vi "data_sim.vi"() -> ()   [LabVIEW 2021]
panel:
  in  "Stop 2":bool
  out "길이 2":i32
  out "연결된 문자열 2":string
  out "CRC-CCITT 2":u16 format="%x"
  out "CRC-CCITT":u16 format="%x"
  out "연결된 문자열":string
  out "길이":i32
  in  "Stop":bool
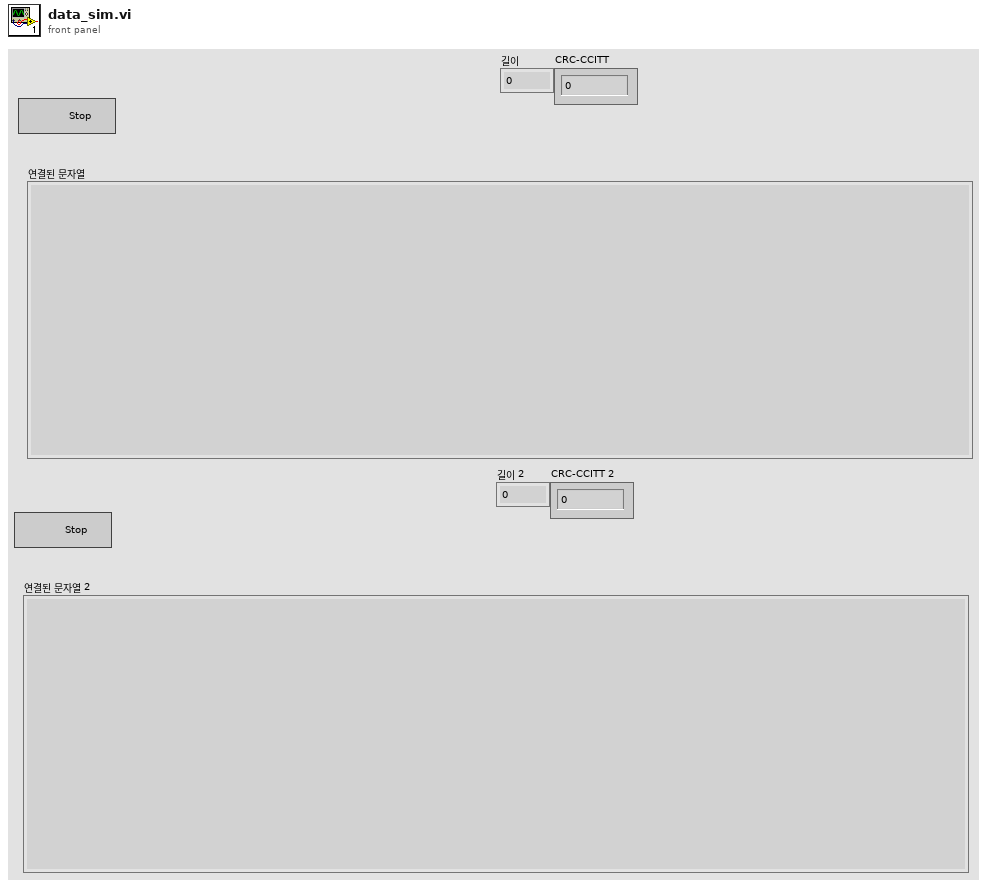
[diagram p1: front panel]
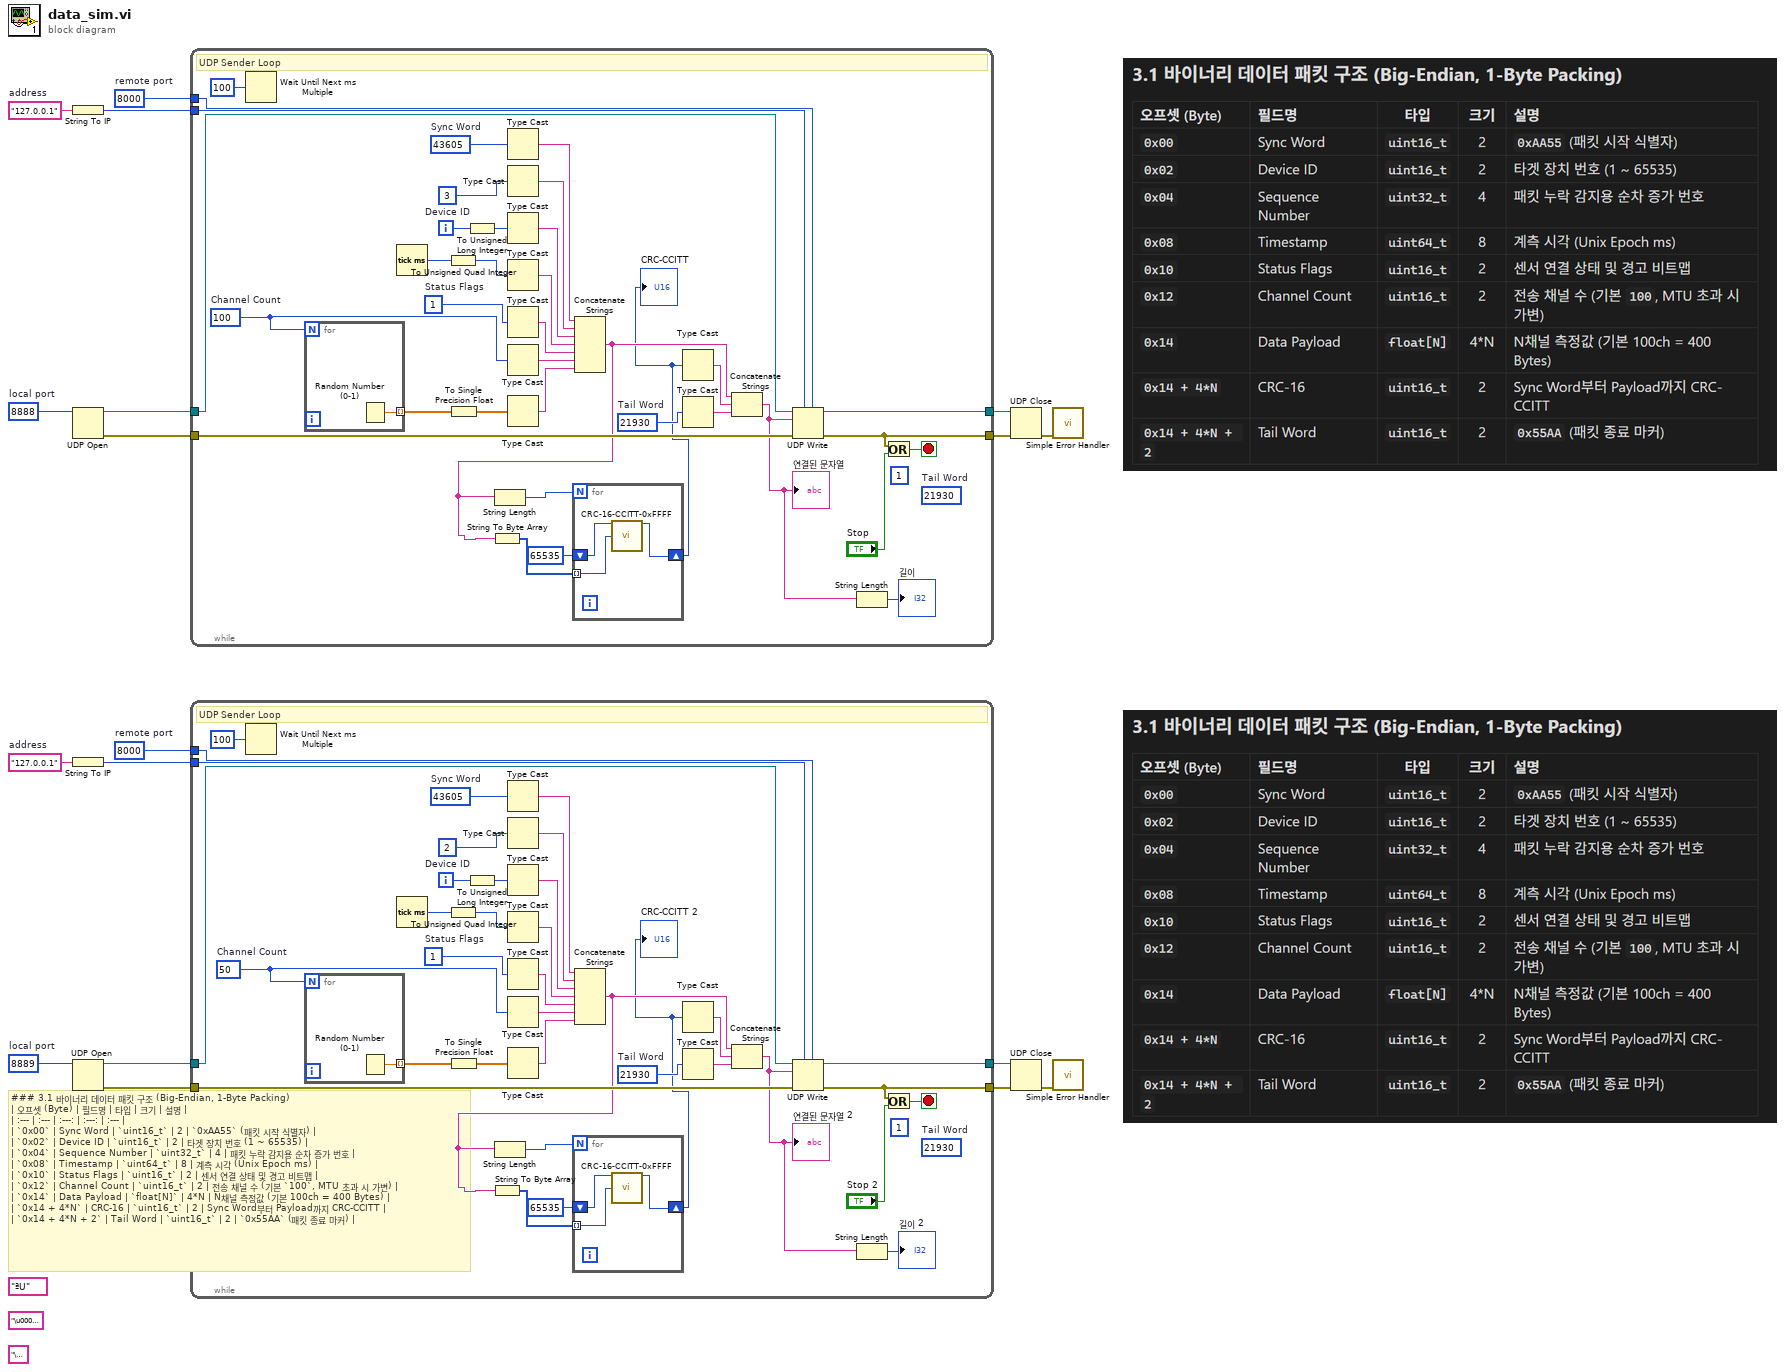
[diagram p0: block diagram]
diagram:
  w9 = u16 8000  # remote port
  w8 = u16 8889  # local port
  w3 = "127.0.0.1"  # address
  (unwired) "\u0001"
  (unwired) "\u0000\u0001"
  (unwired) "ªU"
  w10 = u16 8000  # remote port
  w11 = u16 8888  # local port
  w16 = "127.0.0.1"  # address
  # "### 3.1 바이너리 데이터 패킷 구조 (Big-Endian, 1-Byte Packing)\n| 오프셋 (Byte) | 필드명 | 타입 | 크기 | 설명 |\n| :--- | :--- | :---: | :---: | :--- |\n| `0x00` | Sync Word | `uint16_t` | 2 | `0xAA55` (패킷 시작 식별자) |\n| `0x02` | Device ID | `uint16_t` | 2 | 타겟 장치 번호 (1 ~ 65535) |\n| `0x04` | Sequence Number | `uint32_t` | 4 | 패킷 누락 감지용 순차 증가 번호 |\n| `0x08` | Timestamp | `uint64_t` | 8 | 계측 시각 (Unix Epoch ms) |\n| `0x10` | Status Flags | `uint16_t` | 2 | 센서 연결 상태 및 경고 비트맵 |\n| `0x12` | Channel Count | `uint16_t` | 2 | 전송 채널 수 (기본 `100`, MTU 초과 시 가변) |\n| `0x14` | Data Payload | `float[N]` | 4*N | N채널 측정값 (기본 100ch = 400 Bytes) |\n| `0x14 + 4*N` | CRC-16 | `uint16_t` | 2 | Sync Word부터 Payload까지 CRC-CCITT |\n| `0x14 + 4*N + 2` | Tail Word | `uint16_t` | 2 | `0x55AA` (패킷 종료 마커) |"
  n1 = String To IP(1:w16) -> (0:w14:u32)
  n2 = UDP Open(11:w11) -> (port=w13:refnum<k16>, 0:w12:errorcluster)  [unwired: 4 in, 1 out]
  n3 = String To IP(1:w3) -> (0:w5:u32)
  n4 = UDP Open(11:w8) -> (port=w6:refnum<k16>, 0:w7:errorcluster)  [unwired: 4 in, 1 out]
  n5 = while {
    tunnel: [w49] -> w17
    tunnel: w13 -> [w54]
    tunnel: w12 -> [w53]
    tunnel: [w50] -> w18
    tunnel: w14 -> [w48]
    tunnel: w10 -> [w46]
    i -> [w25]
    stop <- w52 stop-if-true
    w43 = u16 21930  # Tail Word
    (unwired) u16 21930  # Tail Word
    w36 = u16 100  # Channel Count
    w37 = u16 1  # Status Flags
    (unwired) u16 1
    w39 = u16 3  # Device ID
    w40 = u16 43605  # Sync Word
    # "UDP Sender Loop"
    n6 = Wait Until Next ms Multiple(millisecond multiple=u32 100 ("milliseconds to wait")) -> ()  [unwired: 1 out]
    n7 = for {
      N: w36 -> [_]
      tunnel: [w58] -> w44 mode=indexing
      n8 = Random Number (0-1)() -> (number: 0 to 1=w58:dbl)
    }
    n9 = Tick Count (ms)() -> (millisecond timer value=w45:u32)
    n10 = To Unsigned Quad Integer(1:w45) -> (0:w38:u64)
    n11 = To Single Precision Float(number=w44) -> (single precision float=w41:sgl[])
    n12 = To Unsigned Long Integer(number=w25) -> (unsigned 32bit integer=w24:u32)
    n13 = Type Cast(x=w40) -> (*(type *) &x=w30:string)  [unwired: 1 in]
    n14 = Type Cast(x=w39) -> (*(type *) &x=w31:string)  [unwired: 1 in]
    n15 = Type Cast(x=w24) -> (*(type *) &x=w32:string)  [unwired: 1 in]
    n16 = Type Cast(x=w38) -> (*(type *) &x=w33:string)  [unwired: 1 in]
    n17 = Type Cast(x=w37) -> (*(type *) &x=w34:string)  [unwired: 1 in]
    n18 = Type Cast(x=w36) -> (*(type *) &x=w35:string)  [unwired: 1 in]
    n19 = Type Cast(x=w41) -> (*(type *) &x=w27:string)  [unwired: 1 in]
    n20 = Concatenate Strings(w30, w31, w32, w33, w34, w35, w27) -> (w20:string)
    n21 = String To Byte Array(string=w20) -> (unsigned byte array=w23:u8[])
    n22 = String Length(string=w20) -> (length=w22:i32)
    n23 = for {
      N: w22 -> [_]
      tunnel: w23 -> [w56] mode=indexing
      shift-right: [w55] -> w19
      shift-left: u16 65535 ("CRC") -> [w57]
      n24 = call "CRC-16-CCITT-0xFFFF.vi"("CRC In"=w57, "Data"=w56) -> ("CRC"=w55:u16)  [unwired: 12 in, 1 out]
    }
    "CRC-CCITT" <- w19
    n25 = Type Cast(x=w19) -> (*(type *) &x=w29:string)  [unwired: 1 in]
    n26 = Type Cast(x=w43) -> (*(type *) &x=w28:string)  [unwired: 1 in]
    n27 = Concatenate Strings(w20, w29, w28) -> (w26:string)
    "연결된 문자열" <- w26
    n28 = UDP Write(address=w48, port or service name=w46, connection ID=w54, data in=w26, 8:w53) -> (error out=w49:errorcluster, 3:w50:refnum<k16>)  [unwired: 1 in]
    n29 = String Length(string=w26) -> (length=→"길이":i32)
    n30 = Or(x=w49, y="Stop") -> (x .or. y?=w52:bool)
  }
  n31 = while {
    tunnel: [w89] -> w2
    tunnel: w6 -> [w94]
    tunnel: w7 -> [w93]
    tunnel: [w90] -> w1
    tunnel: w5 -> [w88]
    tunnel: w9 -> [w86]
    i -> [w65]
    stop <- w92 stop-if-true
    w83 = u16 21930  # Tail Word
    (unwired) u16 21930  # Tail Word
    w76 = u16 50  # Channel Count
    w77 = u16 1  # Status Flags
    (unwired) u16 1
    w79 = u16 2  # Device ID
    w80 = u16 43605  # Sync Word
    # "UDP Sender Loop"
    n32 = Wait Until Next ms Multiple(millisecond multiple=u32 100 ("milliseconds to wait")) -> ()  [unwired: 1 out]
    n33 = for {
      N: w76 -> [_]
      tunnel: [w98] -> w84 mode=indexing
      n34 = Random Number (0-1)() -> (number: 0 to 1=w98:dbl)
    }
    n35 = Tick Count (ms)() -> (millisecond timer value=w85:u32)
    n36 = To Unsigned Quad Integer(1:w85) -> (0:w78:u64)
    n37 = To Single Precision Float(number=w84) -> (single precision float=w81:sgl[])
    n38 = To Unsigned Long Integer(number=w65) -> (unsigned 32bit integer=w64:u32)
    n39 = Type Cast(x=w80) -> (*(type *) &x=w70:string)  [unwired: 1 in]
    n40 = Type Cast(x=w79) -> (*(type *) &x=w71:string)  [unwired: 1 in]
    n41 = Type Cast(x=w64) -> (*(type *) &x=w72:string)  [unwired: 1 in]
    n42 = Type Cast(x=w78) -> (*(type *) &x=w73:string)  [unwired: 1 in]
    n43 = Type Cast(x=w77) -> (*(type *) &x=w74:string)  [unwired: 1 in]
    n44 = Type Cast(x=w76) -> (*(type *) &x=w75:string)  [unwired: 1 in]
    n45 = Type Cast(x=w81) -> (*(type *) &x=w67:string)  [unwired: 1 in]
    n46 = Concatenate Strings(w70, w71, w72, w73, w74, w75, w67) -> (w60:string)
    n47 = String To Byte Array(string=w60) -> (unsigned byte array=w63:u8[])
    n48 = String Length(string=w60) -> (length=w62:i32)
    n49 = for {
      N: w62 -> [_]
      tunnel: w63 -> [w96] mode=indexing
      shift-right: [w95] -> w59
      shift-left: u16 65535 ("CRC") -> [w97]
      n50 = call "CRC-16-CCITT-0xFFFF.vi"("CRC In"=w97, "Data"=w96) -> ("CRC"=w95:u16)  [unwired: 12 in, 1 out]
    }
    "CRC-CCITT 2" <- w59
    n51 = Type Cast(x=w59) -> (*(type *) &x=w69:string)  [unwired: 1 in]
    n52 = Type Cast(x=w83) -> (*(type *) &x=w68:string)  [unwired: 1 in]
    n53 = Concatenate Strings(w60, w69, w68) -> (w66:string)
    "연결된 문자열 2" <- w66
    n54 = UDP Write(address=w88, port or service name=w86, connection ID=w94, data in=w66, 8:w93) -> (error out=w89:errorcluster, 3:w90:refnum<k16>)  [unwired: 1 in]
    n55 = String Length(string=w66) -> (length=→"길이 2":i32)
    n56 = Or(x=w89, y="Stop 2") -> (x .or. y?=w92:bool)
  }
  n57 = UDP Close(connection ID=w18, 8:w17) -> (error out=w15:errorcluster)  [unwired: 1 out]
  n58 = UDP Close(connection ID=w1, 8:w2) -> (error out=w4:errorcluster)  [unwired: 1 out]
  n59 = call <vilib>:"Simple Error Handler.vi"("error in (no error)"=w15) -> ()  [unwired: 4 in, 5 out]
  n60 = call <vilib>:"Simple Error Handler.vi"("error in (no error)"=w4) -> ()  [unwired: 4 in, 5 out]
